vi "default subpanel.vi"() -> ()   [LabVIEW 2013, in "VI modification.lvclass"]
uses:
  VI modification.lvclass
  <vilib>/NI/Configuration Framework/Node/NodeRef.ctl
  <vilib>/NI/Configuration Framework/Node/NISE_CEF_Node.lvclass
  <vilib>/NI/AMC/Message Queue.ctl
  <vilib>/NI/AMC/Message.ctl
  <vilib>/NI/Tools/Keyed Array/KeyedArray.ctl
  <vilib>/NI/Configuration Framework/Node/UserEventRef.ctl
  <vilib>/NI/Configuration Framework/Controls/EventCluster.ctl
  VI modification.lvclass/VI modification.ctl
  Write exclusions.vi
  Read exclusions.vi
  <vilib>/NI/Tools/Keyed Array/Tools_KeyedArray.lvlib
  <vilib>/NI/AMC/AMC.lvlib
  <vilib>/NI/Configuration Framework/NISE_CEF_TreeControl.lvlib
panel:
  in  "user event":T1
  in  "main queue":T2
  in  "node ref":T3
  in  "exclusions":string[](array[string])
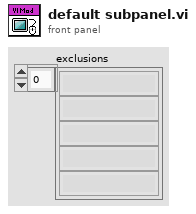
[diagram p1: front panel]
types:
  T1 = typedef "NISE_CEF_Node.lvclass/UserEventRef.ctl" = refnum<user-event>
  T2 = typedef "AMC.lvlib/Message Queue.ctl" = refnum<queue>
  T3 = typedef "NISE_CEF_Node.lvclass/NodeRef.ctl" = refnum<data-value>
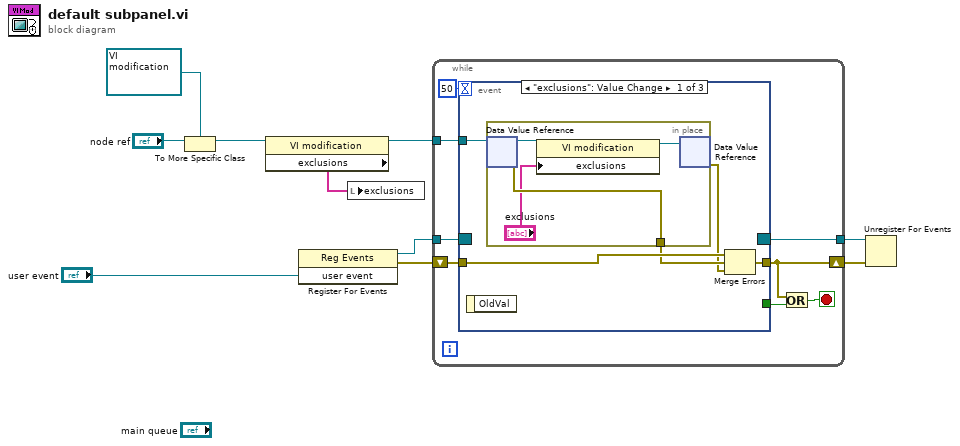
[diagram p0: block diagram]
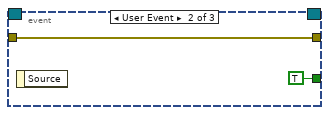
[diagram p2: hidden frame]
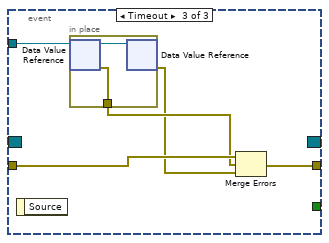
[diagram p3: hidden frame]
diagram:
  n1 = To More Specific Class(target class=refnum<data-value> refnum ("node ref 2"), reference="node ref") -> (specific class reference=w3:refnum<data-value>)  [unwired: 1 in, 1 out]
  n2 = property class="VI modification"(reference=w3) -> (reference out=w6:refnum<data-value>, "exclusions"=w5:string[])  [unwired: 1 in, 1 out]
  n3 = register-events("user event") -> (reference out=w9:refnum<event-registration>, error out=w10:errorcluster)  [unwired: 2 in]
  n4 = local write "exclusions"(w5) -> ()
  n5 = while {
    shift-right: [w11] -> w8
    shift-left: w10 -> [w15]
    tunnel: w9 -> [w18]
    tunnel: [w17] -> w7
    tunnel: w6 -> [w14]
    stop <- w12 stop-if-true
    n6 = event shown="[0] \"exclusions\": Value Change" {
      selector: w18 -> [_ _ _]
      dyn-events: [_ _ _] -> w17
      timeout: 50 -> [_ _ _]
      tunnel: [_ TRUE _] -> w16
      tunnel: [w21 w29 w32] -> w11
      tunnel: w15 -> [w23 w29 w34]
      tunnel: w14 -> [w22 _ w33]
      event "exclusions": Value Change {
        n7 = event-data() -> ()  [unwired: 1 in, 1 out]
        n8 = in-place {
          in-place-border: [w27] -> w20
          n9 = in-place-dvr #1(w22) -> (w26:refnum<class "VI modification.lvclass">, w27:errorcluster)
          n10 = property class="VI modification"(reference=w26, "exclusions"="exclusions") -> (reference out=w25:refnum<class "VI modification.lvclass">)  [unwired: 1 in, 1 out]
          n11 = in-place-dvr #1(w25) -> (w19:errorcluster)  [unwired: 1 out]
        }
        n12 = Merge Errors(w23, w20, w19) -> (w21:errorcluster)
      }
      event User Event {
        n13 = event-data() -> ()  [unwired: 1 in, 1 out]
      }
      event Timeout {
        n14 = event-data() -> ()  [unwired: 1 in, 1 out]
        n15 = in-place {
          in-place-border: [w35] -> w31
          n16 = in-place-dvr #2(w33) -> (w36:refnum<class "VI modification.lvclass">, w35:errorcluster)
          n17 = in-place-dvr #2(w36) -> (w30:errorcluster)  [unwired: 1 out]
        }
        n18 = Merge Errors(w34, w31, w30) -> (w32:errorcluster)
      }
    }
    n19 = Or(x=w11, y=w16) -> (x .or. y?=w12:bool)
  }
  n20 = Unregister For Events(event registration refnum=w7, error in=w8) -> ()  [unwired: 1 out]
